vi "Machine_Etat_M1.vi"() -> ()   [LabVIEW 2017]
uses:
  Commande 1.ctl
  <vilib>/Platform/TimedLoop/XDataNode/timing_clust.ctl
  <vilib>/Platform/TimedLoop/XDataNode/nitl_modes.ctl
  <vilib>/Platform/TimedLoop/XDataNode/wakeup.ctl
  <vilib>/myRIO/Instrument Drivers/Onboard IO/DIO/typedefs/DIO Reference.ctl
  <vilib>/myRIO/Common/Instrument Driver Framework/Utilities/typedefs/myRIO Generic Hardware Reference.ctl
  <vilib>/myRIO/Common/Instrument Driver Framework/Utilities/typedefs/Hardware Version Enum.ctl
  <vilib>/myRIO/Common/Instrument Driver Framework/Utilities/typedefs/myRIO v1.0 Reference.ctl
  <vilib>/myRIO/Common/Instrument Driver Framework/Utilities/typedefs/Generic FPGA Reference.ctl
  <vilib>/myRIO/Common/Instrument Driver Framework/myRIO v1.0/DIO/typedefs/DIO Channels List.ctl
  <vilib>/myRIO/Common/Instrument Driver Framework/myRIO v1.0/DIO/typedefs/DIO Channels Enum.ctl
  <vilib>/userdefined/High Color/nirio_resource_hc.ctl
  enum_bras.ctl
  <vilib>/myRIO/Common/Instrument Driver Framework/Utilities/vis/Is FPGA Ref Available.vi
  <vilib>/myRIO/Common/Instrument Driver Framework/myRIO v1.0/DIO/vis/myRIO v1.1 Open DIO.vi
  <vilib>/myRIO/Instrument Drivers/Onboard IO/DIO/vis/Write.vi
  <vilib>/myRIO/Common/Instrument Driver Framework/Utilities/vis/Validate Channels.vi
  <vilib>/myRIO/Common/Instrument Driver Framework/myRIO v1.0/DIO/vis/myRIO v1.0 Reserve DIO.vi
  <vilib>/myRIO/Common/Instrument Driver Framework/myRIO v1.0/Resource Manager/vis/myRIO v1.0 Reserve Channel List.vi
  <vilib>/myRIO/Common/Instrument Driver Framework/myRIO v1.0/DIO/vis/myRIO v1.0 Build MUX Configuration DIO.vi
  <vilib>/myRIO/Common/Instrument Driver Framework/myRIO v1.0/Resource Manager/vis/myRIO v1.0 Reserve Channel.vi
  <vilib>/myRIO/Common/Instrument Driver Framework/myRIO v1.0/Resource Manager/vis/myRIO v1.0 Unreserve Channel.vi
  <vilib>/myRIO/Common/Instrument Driver Framework/myRIO v1.0/Resource Manager/vis/myRIO v1.0 Create Configuration List.vi
  <vilib>/myRIO/Common/Instrument Driver Framework/myRIO v1.0/Resource Manager/vis/myRIO v1.0 Build Mutex Name.vi
  <vilib>/Utility/VariantDataType/GetNumericInfo.vi
  <vilib>/Utility/error.llb/Error Cluster From Error Code.vi
  <vilib>/myRIO/Common/Instrument Driver Framework/myRIO v1.0/myRIO v1.1 Open.vi
  <vilib>/myRIO/Common/Instrument Driver Framework/Utilities/vis/IO Manager.vi
  <vilib>/myRIO/Common/Instrument Driver Framework/Utilities/vis/Configuration Manager.vi
  <vilib>/myRIO/Common/Instrument Driver Framework/myRIO v1.0/Resource Manager/vis/myRIO v1.0 Configure IO.vi
  <vilib>/myRIO/Common/Instrument Driver Framework/myRIO v1.0/myRIO v1.0 Close.vi
  <vilib>/myRIO/Common/Instrument Driver Framework/myRIO v1.0/DIO/vis/myRIO v1.0 Write DIO.vi
  <vilib>/Platform/TimedLoop/XDataNode/XDataNode.xnode
  <vilib>/myRIO/Express VI/Onboard Devices/LED/LED Express VI.xnode
  <vilib>/myRIO/Instrument Drivers/Onboard IO/DIO/vis/myRIO DIO Open.xnode
  <vilib>/Platform/TimedLoop/XDataNode/XDNodeRunTimeDep.lvlib
  <vilib>/myRIO/Instrument Drivers/Onboard IO/DIO/DIO.lvlib
panel:
  out "Erreur":errorcluster
  out "Vert : dévi à droite 2":bool
  out "Graphe déroulant 2":u32(graph)
  out "x > y ? 2":bool[](array[boolean])
  out "Cluster 3":T1
  out "4 LED droite 2":bool[](array[boolean])
  out "4 LED gauche 2":bool[](array[boolean])
  out "droite 2":u32
  out "gauche 2":u32
  out "Énum 2":T2
  out "seuil":u32
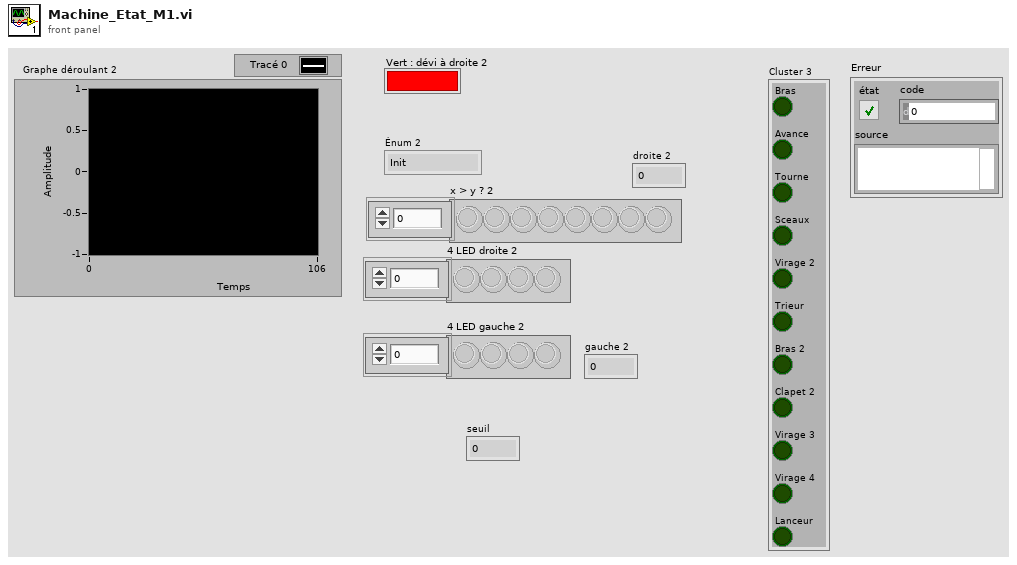
[diagram p1: front panel]
types:
  T1 = typedef "Voyant machine d'état.ctl" = cluster{"Bras":bool, "Avance":bool, "Tourne":bool, "Sceaux":bool, "Virage 2":bool, "Trieur":bool, "Bras 2":bool, "Clapet 2":bool, "Virage 3":bool, "Virage 4":bool, "Lanceur":bool}
  T2 = typedef "Commande 1.ctl" = enum16{"Init", "Bras", "Clapet 1", "Virage 1", "Sceaux 0", "Sceaux 1", "Sceaux 2", "Sceaux 3", "Sceaux 4", "Virage 2", "Recule", "Trieur", "Bras 2", "Intersection", "Clapet 2", "Virage 3", "Virage 4", "Avance", "Lanceur", "End"}
  T3 = typedef "XDNodeRunTimeDep.lvlib/timing_clust.ctl" = cluster{"Expected End [f-1]":u64, "Actual End [f-1]":u64, "Finished Late? [f-1]":bool, "Expected End [i-1]":u64, "Actual End [i-1]":u64, "Finished Late? [i-1]":bool, "Expected Start [i]":u64, "Actual Start [i]":u64, "Expected Start [f]":u64, "Actual Start [f]":u64, "Source Name":string, "Structure Name":string, "Period":i64, "Deadline":i64, "Offset":i64, "Start":i64, "Priority":i32, "Timeout":i32, "Mode":T4, "Wakeup Reason":T5, "Error":errorcluster, "Source Type":string, "Secondary Source Type":string, "Global End Time":u64, "Global Start Time":u64, "Frame Duration":u64, "Iteration Duration":u64, "Assigned CPU":i32, "I/O Scan Engine Mode":u32}
  T4 = typedef "XDNodeRunTimeDep.lvlib/nitl_modes.ctl" = enum32{"No Change", "Process missed periods, maintain original phase", "Discard missed periods, maintain original phase", "Process missed periods, ignore original phase", "Discard missed periods, ignore original phase"}
  T5 = typedef "XDNodeRunTimeDep.lvlib/wakeup.ctl" = enum32{"Normal", "Aborted", "Asynchronous wakeup", "Timing source error", "Timed loop error", "Timeout"}
  T6 = typedef "DIO.lvlib/DIO Reference.ctl" = cluster{"myRIO Reference":T7, "DIO Channels List":T11}
  T7 = typedef "myRIO Generic Hardware Reference.ctl" = cluster{"myRIO Model":T8, "myRIO Hardware Reference":T9}
  T8 = typedef "Hardware Version Enum.ctl" = enum16{"Unknown", "myRIO-1900", "myRIO-1950", "roboRIO", "NI ELVIS RIO CM"}
  T9 = typedef "myRIO v1.0 Reference.ctl" = cluster{"Generic FPGA Reference":T10, "Allow multiple opens":bool}
  T10 = typedef "Generic FPGA Reference.ctl" = refnum<k20>
  T11 = typedef "DIO Channels List.ctl" = T12[]
  T12 = typedef "DIO Channels Enum.ctl" = enum16{"Not Connected", "C/DIO0", "C/DIO1", "C/DIO2", "C/DIO3", "C/DIO4", "C/DIO5", "C/DIO6", "C/DIO7", "A/DIO0", "A/DIO1", "A/DIO2", "A/DIO3", "A/DIO4", "A/DIO5", "A/DIO6", "A/DIO7", "A/DIO8", "A/DIO9", "A/DIO10", "A/DIO11", "A/DIO12", "A/DIO13", "A/DIO14", "A/DIO15", "B/DIO0", "B/DIO1", "B/DIO2", "B/DIO3", "B/DIO4", "B/DIO5", "B/DIO6", "B/DIO7", "B/DIO8", "B/DIO9", "B/DIO10", "B/DIO11", "B/DIO12", "B/DIO13", "B/DIO14", "B/DIO15", "LED0", "LED1", "LED2", "LED3", "Button0", "DIO/DIO0", "DIO/DIO1", "DIO/DIO2", "DIO/DIO3", "DIO/DIO4", "DIO/DIO5", "DIO/DIO6", "DIO/DIO7", "DIO/DIO8", "DIO/DIO9", "SPI/CS0", "SPI/CS1", "SPI/CS2", "SPI/CS3", "LED RADIO (Green)", "LED RADIO (Red)", "LED COMM (Green)", "LED COMM (Red)", "LED MODE (Green)", "LED MODE (Red)"}
  T13 = typedef "nirio_resource_hc.ctl" = tag
  T14 = typedef "enum_bras.ctl" = enum16{"Depart Bras", "Clapet Bras", "Inactif Bras", "Seaux Bras"}
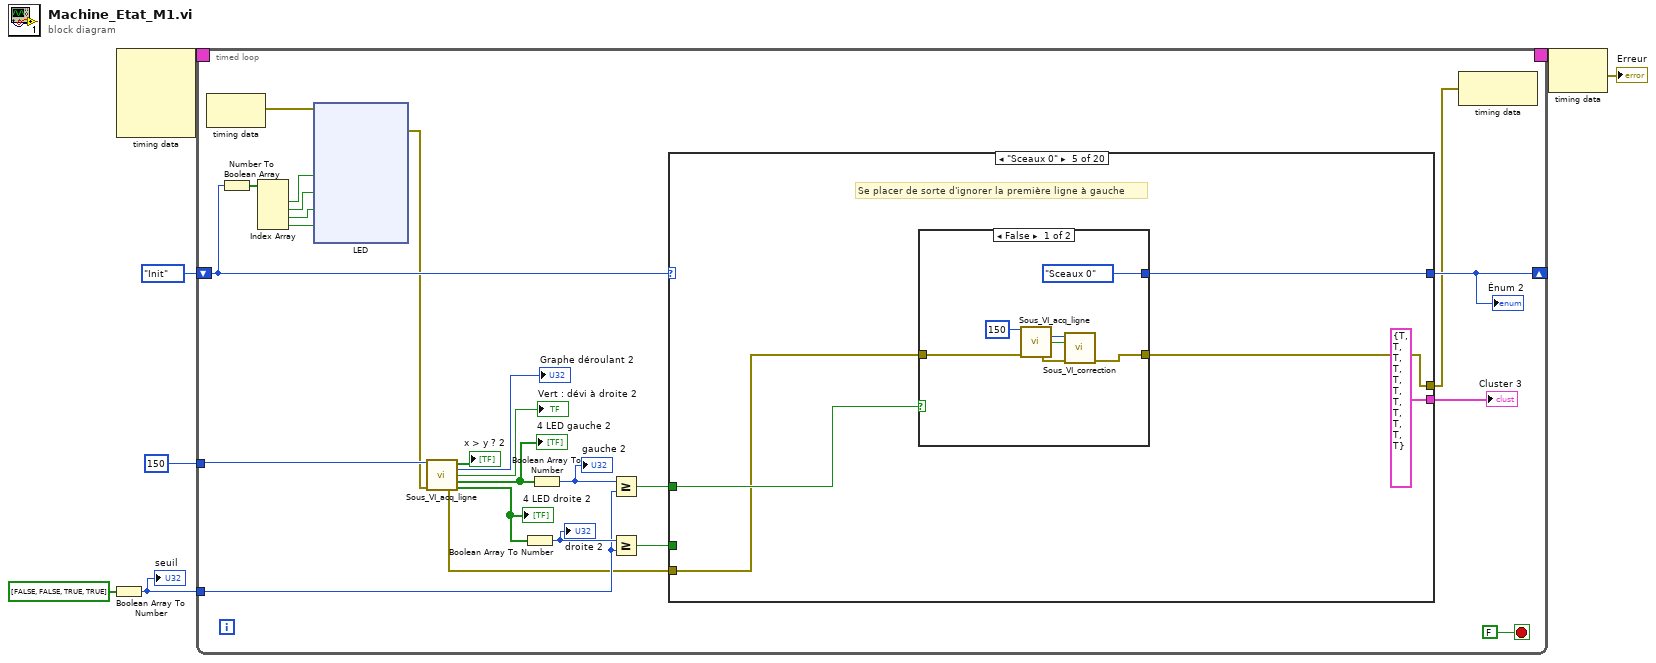
[diagram p0: block diagram]
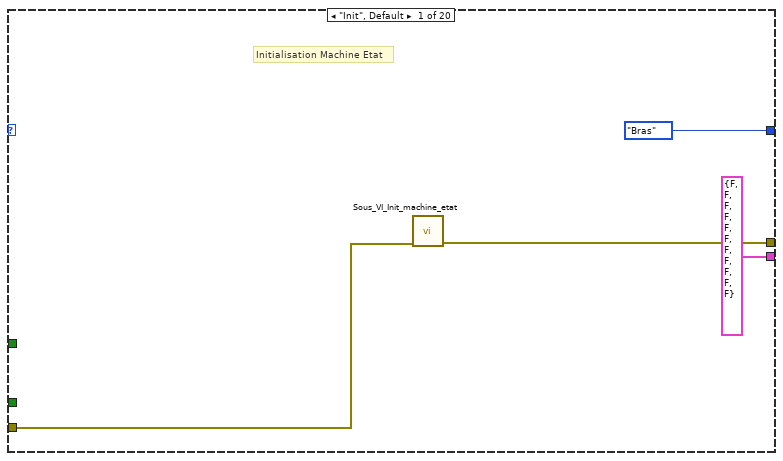
[diagram p2: hidden frame]
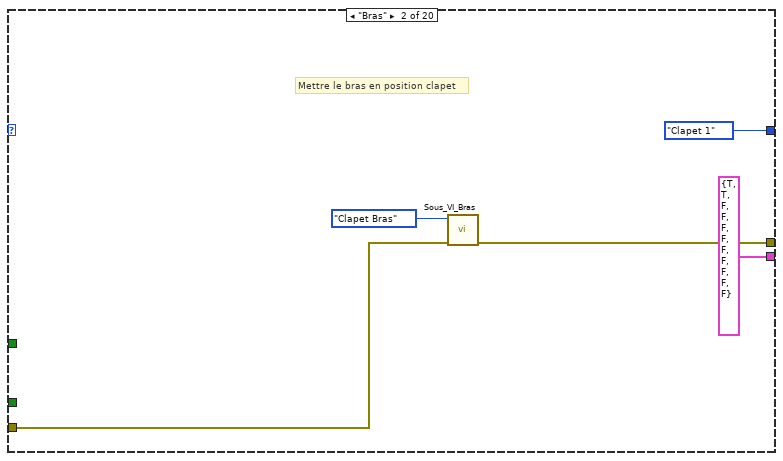
[diagram p3: hidden frame]
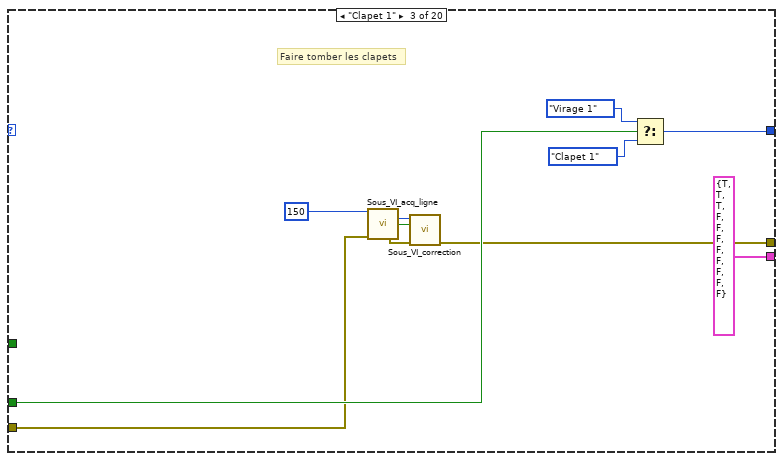
[diagram p4: hidden frame]
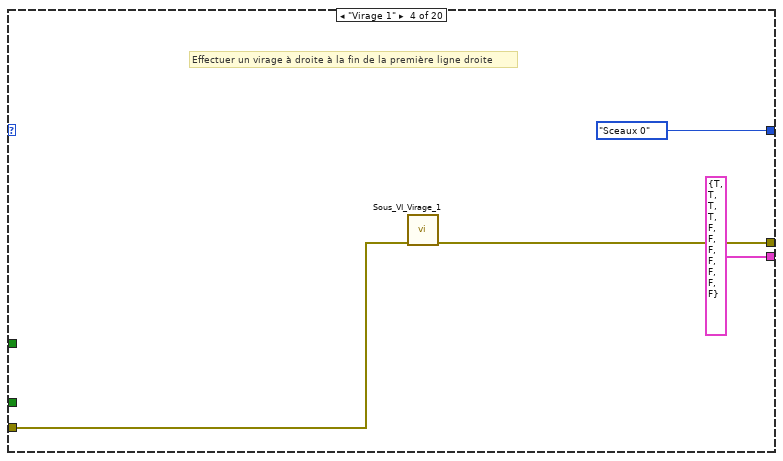
[diagram p5: hidden frame]
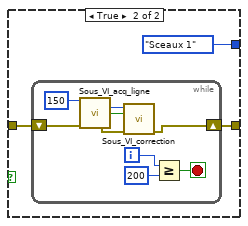
[diagram p6: hidden frame]
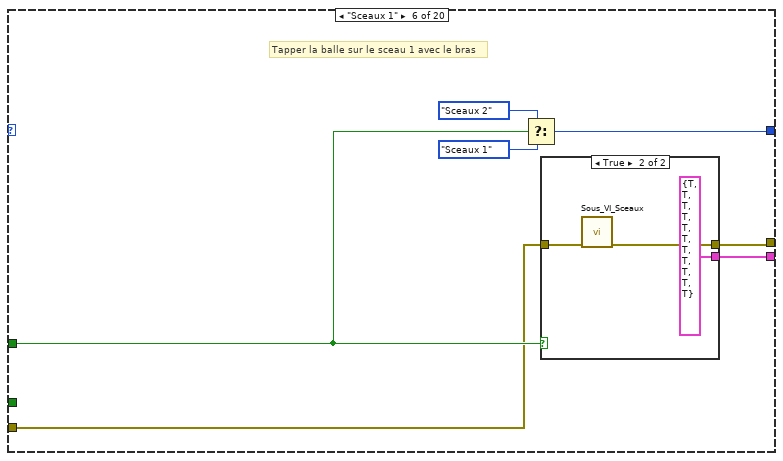
[diagram p7: hidden frame]
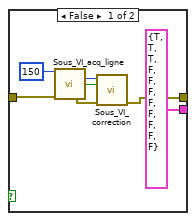
[diagram p8: hidden frame]
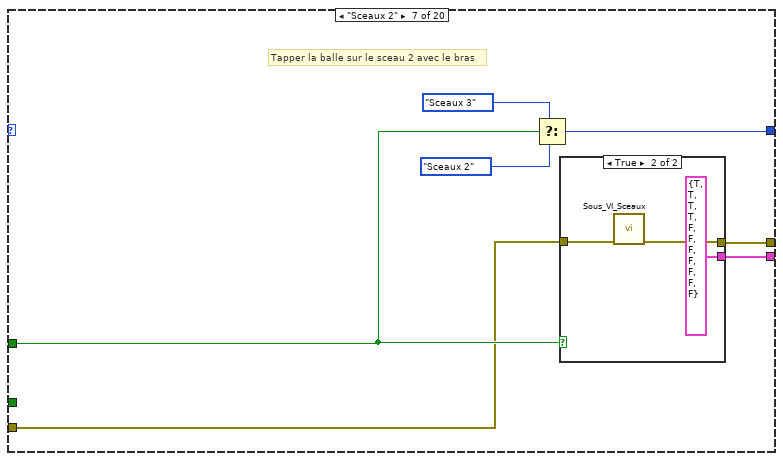
[diagram p9: hidden frame]
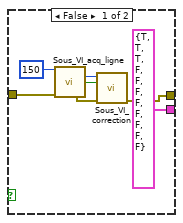
[diagram p10: hidden frame]
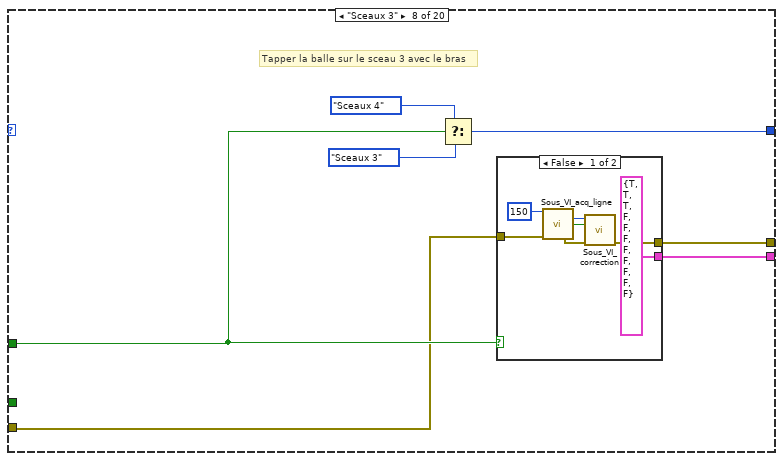
[diagram p11: hidden frame]
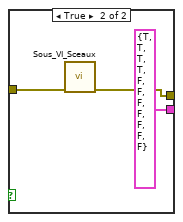
[diagram p12: hidden frame]
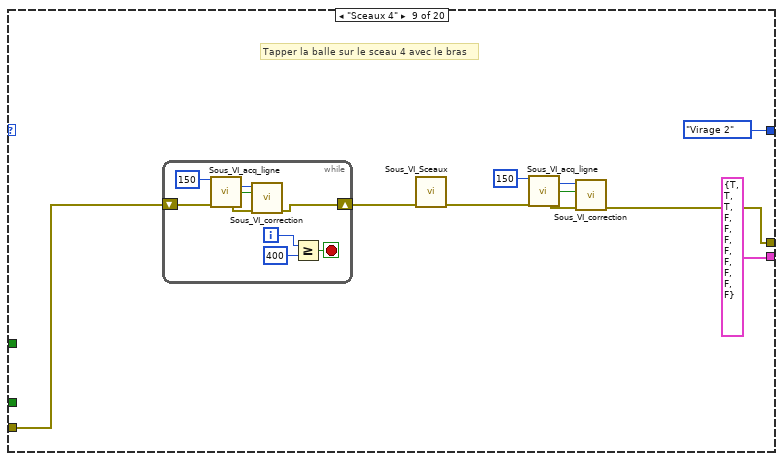
[diagram p13: hidden frame]
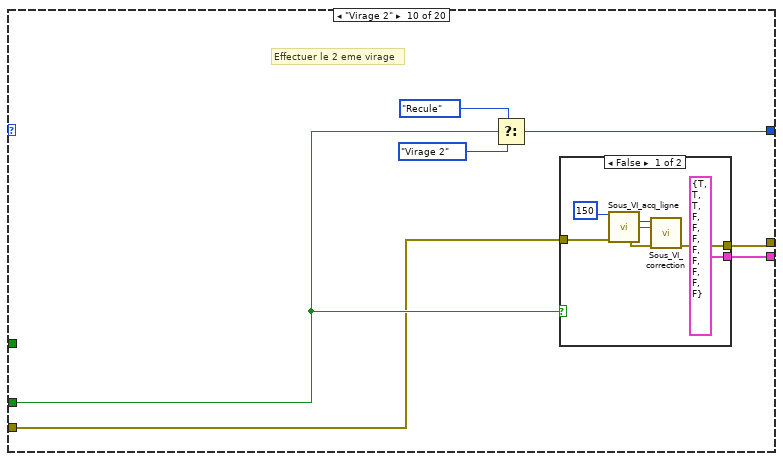
[diagram p14: hidden frame]
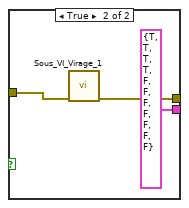
[diagram p15: hidden frame]
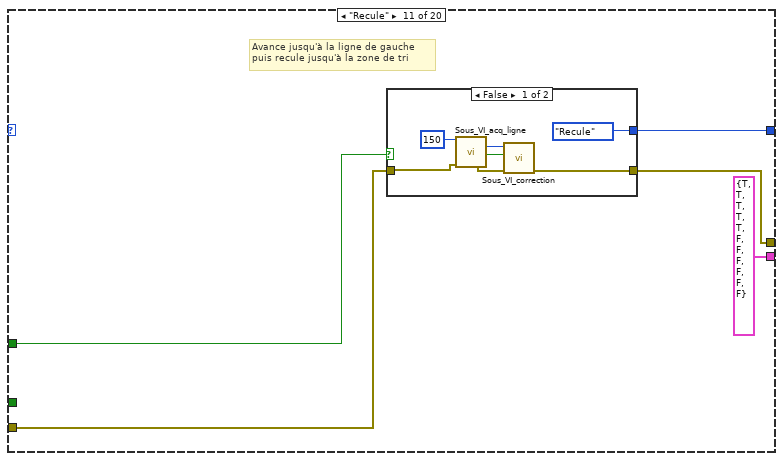
[diagram p16: hidden frame]
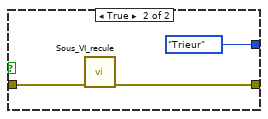
[diagram p17: hidden frame]
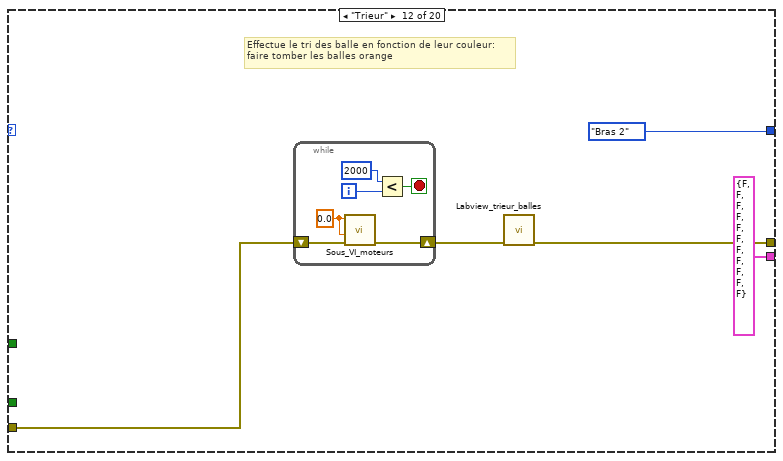
[diagram p18: hidden frame]
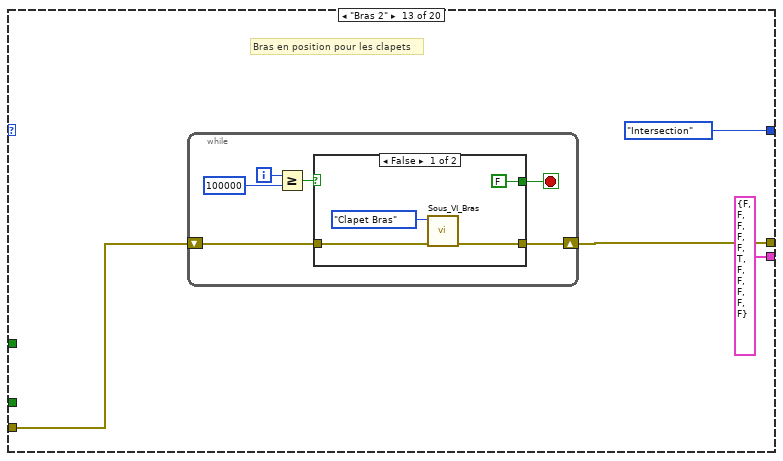
[diagram p19: hidden frame]
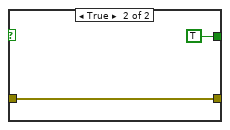
[diagram p20: hidden frame]
diagram:
  n1 = Boolean Array To Number(Boolean array=bool[] [FALSE, FALSE, TRUE, TRUE] ("x < y ? 2")) -> (number=w3:u32)
  "seuil" <- w3
  n2 = node-c288() -> (w6:T3)  [unwired: 4 in]
  n3 = timed-loop {
    tunnel: 150 ("value") -> [w26]
    shift-right: [w31] -> _
    shift-left: Commande_1."Init" -> [w18]
    tunnel: w3 -> [w20]
    timing: w6 -> [_]
    timing-out: [_] -> w5
    stop <- FALSE stop-if-true
    n4 = node-c288() -> (w11:errorcluster)  [unwired: 1 in]
    n5 = Number To Boolean Array(number=w18) -> (Boolean array=w17:bool[])
    n6 = Index Array(array=w17) -> (element #1=w16:bool, element #2=w15:bool, element #3=w12:bool, element #4=w14:bool)  [unwired: 4 in]
    n7 = xnode "LED"("LED0"=w16, "LED1"=w15, "LED2"=w12, "LED3"=w14, "error in (no error)"=w11) -> ("error out"=w10:errorcluster)
    n8 = call "Sous_VI_acq_ligne.vi"("Seuil"=w26, "error in (no error)"=w10) -> ("x > y ?"=→"x > y ? 2":bool[], "Décalage"=→"Graphe déroulant 2":u32, "G/D ?"=→"Vert : dévi à droite 2":bool, "4 LED gauches"=w23:bool[], "error out"=w9:errorcluster, "4 LED droite"=w22:bool[])  [unwired: 8 in]
    "4 LED droite 2" <- w22
    "4 LED gauche 2" <- w23
    n9 = Boolean Array To Number(Boolean array=w22) -> (number=w21:u32)
    "droite 2" <- w21
    n10 = Boolean Array To Number(Boolean array=w23) -> (number=w19:u32)
    "gauche 2" <- w19
    n11 = Greater Or Equal?(x=w19, y=w20) -> (x >= y?=w29:bool)
    n12 = Greater Or Equal?(x=w21, y=w20) -> (x >= y?=w30:bool)
    n13 = case shown="\"Sceaux 0\"" w18 {
      tunnel: [Commande_1."Bras" Commande_1."Clapet 1" w92 Commande_1."Sceaux 0" w103 w127 w144 w160 Commande_1."Virage 2" w196 w212 Commande_1."Bras 2" Commande_1."Intersection" w257 w268 Commande_1."Avance" w305 Commande_1."Lanceur" Commande_1."End" Commande_1."End"] -> w31
      tunnel: w30 -> [_ _ w91 _ _ _ _ _ _ w195 _ _ _ _ w267 _ w304 _ _ _]
      tunnel: [T1 {"Bras"=FALSE, "Avance"=FALSE, "Tourne"=FALSE, "Sceaux"=FALSE, "Virage 2"=FALSE, "Trieur"=FALSE, "Bras 2"=FALSE, "Clapet 2"=FALSE, "Virage 3"=FALSE, "Virage 4"=FALSE, "Lanceur"=FALSE} ("Cluster 2") T1 {"Bras"=TRUE, "Avance"=TRUE, "Tourne"=FALSE, "Sceaux"=FALSE, "Virage 2"=FALSE, "Trieur"=FALSE, "Bras 2"=FALSE, "Clapet 2"=FALSE, "Virage 3"=FALSE, "Virage 4"=FALSE, "Lanceur"=FALSE} ("Cluster 2") T1 {"Bras"=TRUE, "Avance"=TRUE, "Tourne"=TRUE, "Sceaux"=FALSE, "Virage 2"=FALSE, "Trieur"=FALSE, "Bras 2"=FALSE, "Clapet 2"=FALSE, "Virage 3"=FALSE, "Virage 4"=FALSE, "Lanceur"=FALSE} ("Cluster 2") T1 {"Bras"=TRUE, "Avance"=TRUE, "Tourne"=TRUE, "Sceaux"=TRUE, "Virage 2"=FALSE, "Trieur"=FALSE, "Bras 2"=FALSE, "Clapet 2"=FALSE, "Virage 3"=FALSE, "Virage 4"=FALSE, "Lanceur"=FALSE} ("Cluster 2") T1 {"Bras"=TRUE, "Avance"=TRUE, "Tourne"=TRUE, "Sceaux"=TRUE, "Virage 2"=TRUE, "Trieur"=TRUE, "Bras 2"=TRUE, "Clapet 2"=TRUE, "Virage 3"=TRUE, "Virage 4"=TRUE, "Lanceur"=TRUE} ("Cluster 2") w126 w146 w163 T1 {"Bras"=TRUE, "Avance"=TRUE, "Tourne"=TRUE, "Sceaux"=FALSE, "Virage 2"=FALSE, "Trieur"=FALSE, "Bras 2"=FALSE, "Clapet 2"=FALSE, "Virage 3"=FALSE, "Virage 4"=FALSE, "Lanceur"=FALSE} ("Cluster 2") w199 T1 {"Bras"=TRUE, "Avance"=TRUE, "Tourne"=TRUE, "Sceaux"=TRUE, "Virage 2"=TRUE, "Trieur"=FALSE, "Bras 2"=FALSE, "Clapet 2"=FALSE, "Virage 3"=FALSE, "Virage 4"=FALSE, "Lanceur"=FALSE} ("Cluster 2") T1 {"Bras"=FALSE, "Avance"=FALSE, "Tourne"=FALSE, "Sceaux"=FALSE, "Virage 2"=FALSE, "Trieur"=FALSE, "Bras 2"=FALSE, "Clapet 2"=FALSE, "Virage 3"=FALSE, "Virage 4"=FALSE, "Lanceur"=FALSE} ("Cluster 2") T1 {"Bras"=FALSE, "Avance"=FALSE, "Tourne"=FALSE, "Sceaux"=FALSE, "Virage 2"=FALSE, "Trieur"=TRUE, "Bras 2"=FALSE, "Clapet 2"=FALSE, "Virage 3"=FALSE, "Virage 4"=FALSE, "Lanceur"=FALSE} ("Cluster 2") T1 {"Bras"=FALSE, "Avance"=FALSE, "Tourne"=FALSE, "Sceaux"=FALSE, "Virage 2"=FALSE, "Trieur"=TRUE, "Bras 2"=TRUE, "Clapet 2"=FALSE, "Virage 3"=FALSE, "Virage 4"=FALSE, "Lanceur"=FALSE} ("Cluster 2") T1 {"Bras"=FALSE, "Avance"=FALSE, "Tourne"=FALSE, "Sceaux"=FALSE, "Virage 2"=FALSE, "Trieur"=TRUE, "Bras 2"=TRUE, "Clapet 2"=FALSE, "Virage 3"=FALSE, "Virage 4"=FALSE, "Lanceur"=FALSE} ("Cluster 2") T1 {"Bras"=FALSE, "Avance"=FALSE, "Tourne"=FALSE, "Sceaux"=FALSE, "Virage 2"=FALSE, "Trieur"=TRUE, "Bras 2"=TRUE, "Clapet 2"=TRUE, "Virage 3"=TRUE, "Virage 4"=FALSE, "Lanceur"=FALSE} ("Cluster 2") T1 {"Bras"=FALSE, "Avance"=FALSE, "Tourne"=FALSE, "Sceaux"=FALSE, "Virage 2"=FALSE, "Trieur"=FALSE, "Bras 2"=TRUE, "Clapet 2"=TRUE, "Virage 3"=TRUE, "Virage 4"=TRUE, "Lanceur"=FALSE} ("Cluster 2") T1 {"Bras"=FALSE, "Avance"=FALSE, "Tourne"=FALSE, "Sceaux"=FALSE, "Virage 2"=FALSE, "Trieur"=TRUE, "Bras 2"=TRUE, "Clapet 2"=TRUE, "Virage 3"=TRUE, "Virage 4"=TRUE, "Lanceur"=FALSE} ("Cluster 2") T1 {"Bras"=FALSE, "Avance"=FALSE, "Tourne"=FALSE, "Sceaux"=FALSE, "Virage 2"=FALSE, "Trieur"=FALSE, "Bras 2"=TRUE, "Clapet 2"=TRUE, "Virage 3"=TRUE, "Virage 4"=TRUE, "Lanceur"=TRUE} ("Cluster 2") T1 {"Bras"=FALSE, "Avance"=FALSE, "Tourne"=FALSE, "Sceaux"=FALSE, "Virage 2"=FALSE, "Trieur"=FALSE, "Bras 2"=FALSE, "Clapet 2"=FALSE, "Virage 3"=FALSE, "Virage 4"=FALSE, "Lanceur"=FALSE} ("Cluster 2")] -> w25
      tunnel: w29 -> [_ _ _ _ w102 w125 w143 w159 _ _ w213 _ _ w258 _ _ _ _ _ _]
      tunnel: w9 -> [w75 w80 w84 w95 w100 w124 w141 w158 w181 w194 w211 w227 w237 w252 w263 w277 w298 w309 w313 w317]
      tunnel: [w76 w79 w86 w96 w99 w123 w140 w157 w178 w193 w210 w225 w236 w254 w265 w274 w300 w310 w314 w317] -> w8
      frame "Init", Default {
        # "Initialisation Machine Etat"
        n14 = call "Sous_VI_Init_machine_etat.vi"("error in (no error)"=w75) -> ("error out"=w76:errorcluster)  [unwired: 10 in]
      }
      frame "Bras" {
        # "Mettre le bras en position clapet"
        n15 = call "Sous_VI_Bras.vi"("error in (no error)"=w80, "Enum bras"=enum_bras."Clapet Bras") -> ("error out"=w79:errorcluster)  [unwired: 9 in]
      }
      frame "Clapet 1" {
        # "Faire tomber les clapets"
        n16 = call "Sous_VI_acq_ligne.vi"("Seuil"=150, "error in (no error)"=w84) -> ("Décalage"=w89:u32, "G/D ?"=w87:bool, "error out"=w85:errorcluster)  [unwired: 8 in, 3 out]
        n17 = call "Sous_VI_correction.vi"("error in (no error)"=w85, "G/D ?"=w87, "Décalage"=w89) -> ("error out"=w86:errorcluster)  [unwired: 8 in]
        n18 = Select(t=Commande_1."Virage 1", s=w91, f=Commande_1."Clapet 1") -> (s? t:f=w92:T2)
      }
      frame "Virage 1" {
        # "Effectuer un virage à droite à la fin de la première ligne droite"
        n19 = call "Sous_VI_Virage_1.vi"("error in (no error)"=w95) -> ("error out"=w96:errorcluster)  [unwired: 10 in]
      }
      frame "Sceaux 0" {
        # "Se placer de sorte d'ignorer la première ligne à gauche"
        n20 = case shown="False" w102 {
          tunnel: [Commande_1."Sceaux 0" Commande_1."Sceaux 1"] -> w103
          tunnel: w100 -> [w104 w112]
          tunnel: [w106 w111] -> w99
          frame False {
            n21 = call "Sous_VI_acq_ligne.vi"("Seuil"=150, "error in (no error)"=w104) -> ("Décalage"=w109:u32, "G/D ?"=w107:bool, "error out"=w105:errorcluster)  [unwired: 8 in, 3 out]
            n22 = call "Sous_VI_correction.vi"("error in (no error)"=w105, "G/D ?"=w107, "Décalage"=w109) -> ("error out"=w106:errorcluster)  [unwired: 8 in]
          }
          frame True {
            n23 = while {
              shift-right: [w114] -> w111
              shift-left: w112 -> [w116]
              i -> [w122]
              stop <- w118 stop-if-true
              n24 = call "Sous_VI_acq_ligne.vi"("Seuil"=150, "error in (no error)"=w116) -> ("Décalage"=w120:u32, "G/D ?"=w117:bool, "error out"=w115:errorcluster)  [unwired: 8 in, 3 out]
              n25 = call "Sous_VI_correction.vi"("error in (no error)"=w115, "G/D ?"=w117, "Décalage"=w120) -> ("error out"=w114:errorcluster)  [unwired: 8 in]
              n26 = Greater Or Equal?(x=w122, y=200) -> (x >= y?=w118:bool)
            }
          }
        }
      }
      frame "Sceaux 1" {
        # "Tapper la balle sur le sceau 1 avec le bras"
        n27 = Select(t=Commande_1."Sceaux 2", s=w125, f=Commande_1."Sceaux 1") -> (s? t:f=w127:T2)
        n28 = case shown="True" w125 {
          tunnel: [T1 {"Bras"=TRUE, "Avance"=TRUE, "Tourne"=TRUE, "Sceaux"=FALSE, "Virage 2"=FALSE, "Trieur"=FALSE, "Bras 2"=FALSE, "Clapet 2"=FALSE, "Virage 3"=FALSE, "Virage 4"=FALSE, "Lanceur"=FALSE} ("Cluster 2") T1 {"Bras"=TRUE, "Avance"=TRUE, "Tourne"=TRUE, "Sceaux"=TRUE, "Virage 2"=TRUE, "Trieur"=TRUE, "Bras 2"=TRUE, "Clapet 2"=TRUE, "Virage 3"=TRUE, "Virage 4"=TRUE, "Lanceur"=TRUE} ("Cluster 2")] -> w126
          tunnel: w124 -> [w132 w138]
          tunnel: [w130 w137] -> w123
          frame False {
            n29 = call "Sous_VI_acq_ligne.vi"("Seuil"=150, "error in (no error)"=w132) -> ("Décalage"=w135:u32, "G/D ?"=w133:bool, "error out"=w131:errorcluster)  [unwired: 8 in, 3 out]
            n30 = call "Sous_VI_correction.vi"("error in (no error)"=w131, "G/D ?"=w133, "Décalage"=w135) -> ("error out"=w130:errorcluster)  [unwired: 8 in]
          }
          frame True {
            n31 = call "Sous_VI_Sceaux.vi"("error in (no error)"=w138) -> ("error out"=w137:errorcluster)  [unwired: 10 in]
          }
        }
      }
      frame "Sceaux 2" {
        # "Tapper la balle sur le sceau 2 avec le bras"
        n32 = Select(t=Commande_1."Sceaux 3", s=w143, f=Commande_1."Sceaux 2") -> (s? t:f=w144:T2)
        n33 = case shown="True" w143 {
          tunnel: [T1 {"Bras"=TRUE, "Avance"=TRUE, "Tourne"=TRUE, "Sceaux"=FALSE, "Virage 2"=FALSE, "Trieur"=FALSE, "Bras 2"=FALSE, "Clapet 2"=FALSE, "Virage 3"=FALSE, "Virage 4"=FALSE, "Lanceur"=FALSE} ("Cluster 2") T1 {"Bras"=TRUE, "Avance"=TRUE, "Tourne"=TRUE, "Sceaux"=TRUE, "Virage 2"=FALSE, "Trieur"=FALSE, "Bras 2"=FALSE, "Clapet 2"=FALSE, "Virage 3"=FALSE, "Virage 4"=FALSE, "Lanceur"=FALSE} ("Cluster 2")] -> w146
          tunnel: w141 -> [w149 w155]
          tunnel: [w147 w154] -> w140
          frame False {
            n34 = call "Sous_VI_acq_ligne.vi"("Seuil"=150, "error in (no error)"=w149) -> ("Décalage"=w152:u32, "G/D ?"=w150:bool, "error out"=w148:errorcluster)  [unwired: 8 in, 3 out]
            n35 = call "Sous_VI_correction.vi"("error in (no error)"=w148, "G/D ?"=w150, "Décalage"=w152) -> ("error out"=w147:errorcluster)  [unwired: 8 in]
          }
          frame True {
            n36 = call "Sous_VI_Sceaux.vi"("error in (no error)"=w155) -> ("error out"=w154:errorcluster)  [unwired: 10 in]
          }
        }
      }
      frame "Sceaux 3" {
        # "Tapper la balle sur le sceau 3 avec le bras"
        n37 = Select(t=Commande_1."Sceaux 4", s=w159, f=Commande_1."Sceaux 3") -> (s? t:f=w160:T2)
        n38 = case shown="False" w159 {
          tunnel: [T1 {"Bras"=TRUE, "Avance"=TRUE, "Tourne"=TRUE, "Sceaux"=FALSE, "Virage 2"=FALSE, "Trieur"=FALSE, "Bras 2"=FALSE, "Clapet 2"=FALSE, "Virage 3"=FALSE, "Virage 4"=FALSE, "Lanceur"=FALSE} ("Cluster 2") T1 {"Bras"=TRUE, "Avance"=TRUE, "Tourne"=TRUE, "Sceaux"=TRUE, "Virage 2"=FALSE, "Trieur"=FALSE, "Bras 2"=FALSE, "Clapet 2"=FALSE, "Virage 3"=FALSE, "Virage 4"=FALSE, "Lanceur"=FALSE} ("Cluster 2")] -> w163
          tunnel: w158 -> [w166 w172]
          tunnel: [w164 w171] -> w157
          frame False {
            n39 = call "Sous_VI_acq_ligne.vi"("Seuil"=150, "error in (no error)"=w166) -> ("Décalage"=w169:u32, "G/D ?"=w167:bool, "error out"=w165:errorcluster)  [unwired: 8 in, 3 out]
            n40 = call "Sous_VI_correction.vi"("error in (no error)"=w165, "G/D ?"=w167, "Décalage"=w169) -> ("error out"=w164:errorcluster)  [unwired: 8 in]
          }
          frame True {
            n41 = call "Sous_VI_Sceaux.vi"("error in (no error)"=w172) -> ("error out"=w171:errorcluster)  [unwired: 10 in]
          }
        }
      }
      frame "Sceaux 4" {
        # "Tapper la balle sur le sceau 4 avec le bras"
        n42 = while {
          shift-right: [w184] -> w180
          shift-left: w181 -> [w186]
          i -> [w192]
          stop <- w188 stop-if-true
          n43 = call "Sous_VI_acq_ligne.vi"("Seuil"=150, "error in (no error)"=w186) -> ("Décalage"=w190:u32, "G/D ?"=w187:bool, "error out"=w185:errorcluster)  [unwired: 8 in, 3 out]
          n44 = call "Sous_VI_correction.vi"("error in (no error)"=w185, "G/D ?"=w187, "Décalage"=w190) -> ("error out"=w184:errorcluster)  [unwired: 8 in]
          n45 = Greater Or Equal?(x=w192, y=400) -> (x >= y?=w188:bool)
        }
        n46 = call "Sous_VI_Sceaux.vi"("error in (no error)"=w180) -> ("error out"=w179:errorcluster)  [unwired: 10 in]
        n47 = call "Sous_VI_acq_ligne.vi"("Seuil"=150, "error in (no error)"=w179) -> ("Décalage"=w177:u32, "G/D ?"=w175:bool, "error out"=w174:errorcluster)  [unwired: 8 in, 3 out]
        n48 = call "Sous_VI_correction.vi"("error in (no error)"=w174, "G/D ?"=w175, "Décalage"=w177) -> ("error out"=w178:errorcluster)  [unwired: 8 in]
      }
      frame "Virage 2" {
        # "Effectuer le 2 eme virage"
        n49 = Select(t=Commande_1."Recule", s=w195, f=Commande_1."Virage 2") -> (s? t:f=w196:T2)
        n50 = case shown="False" w195 {
          tunnel: [T1 {"Bras"=TRUE, "Avance"=TRUE, "Tourne"=TRUE, "Sceaux"=FALSE, "Virage 2"=FALSE, "Trieur"=FALSE, "Bras 2"=FALSE, "Clapet 2"=FALSE, "Virage 3"=FALSE, "Virage 4"=FALSE, "Lanceur"=FALSE} ("Cluster 2") T1 {"Bras"=TRUE, "Avance"=TRUE, "Tourne"=TRUE, "Sceaux"=TRUE, "Virage 2"=FALSE, "Trieur"=FALSE, "Bras 2"=FALSE, "Clapet 2"=FALSE, "Virage 3"=FALSE, "Virage 4"=FALSE, "Lanceur"=FALSE} ("Cluster 2")] -> w199
          tunnel: w194 -> [w202 w208]
          tunnel: [w200 w207] -> w193
          frame False {
            n51 = call "Sous_VI_acq_ligne.vi"("Seuil"=150, "error in (no error)"=w202) -> ("Décalage"=w205:u32, "G/D ?"=w203:bool, "error out"=w201:errorcluster)  [unwired: 8 in, 3 out]
            n52 = call "Sous_VI_correction.vi"("error in (no error)"=w201, "G/D ?"=w203, "Décalage"=w205) -> ("error out"=w200:errorcluster)  [unwired: 8 in]
          }
          frame True {
            n53 = call "Sous_VI_Virage_1.vi"("error in (no error)"=w208) -> ("error out"=w207:errorcluster)  [unwired: 10 in]
          }
        }
      }
      frame "Recule" {
        # "Avance jusqu'à la ligne de gauche \npuis recule jusqu'à la zone de tri"
        n54 = case shown="False" w213 {
          tunnel: [Commande_1."Recule" Commande_1."Trieur"] -> w212
          tunnel: w211 -> [w215 w223]
          tunnel: [w216 w222] -> w210
          frame False {
            n55 = call "Sous_VI_acq_ligne.vi"("Seuil"=150, "error in (no error)"=w215) -> ("Décalage"=w219:u32, "G/D ?"=w218:bool, "error out"=w217:errorcluster)  [unwired: 8 in, 3 out]
            n56 = call "Sous_VI_correction.vi"("error in (no error)"=w217, "G/D ?"=w218, "Décalage"=w219) -> ("error out"=w216:errorcluster)  [unwired: 8 in]
          }
          frame True {
            n57 = call "Sous_VI_recule.vi"("error in (no error)"=w223) -> ("error out"=w222:errorcluster)  [unwired: 10 in]
          }
        }
      }
      frame "Trieur" {
        # "Effectue le tri des balle en fonction de leur couleur:\nfaire tomber les balles orange"
        n58 = while {
          shift-right: [w230] -> w226
          shift-left: w227 -> [w231]
          i -> [w235]
          stop <- w233 stop-if-true
          w232 = 0.0 ("moteur gauche vite")
          n59 = call "Sous_VI_moteurs.vi"("error in (no error)"=w231, "Moteur Droit"=w232, "Moteur Gauche"=w232) -> ("error out"=w230:errorcluster)  [unwired: 8 in]
          n60 = Less?(x=2000, y=w235) -> (x < y?=w233:bool)
        }
        n61 = call "Labview_trieur_balles.vi"("error in (no error)"=w226) -> ("error out"=w225:errorcluster)  [unwired: 10 in]
      }
      frame "Bras 2" {
        # "Bras en position pour les clapets"
        n62 = while {
          shift-right: [w240] -> w236
          shift-left: w237 -> [w241]
          i -> [w242]
          stop <- w244 stop-if-true
          n63 = Greater Or Equal?(x=w242, y=100000) -> (x >= y?=w245:bool)
          n64 = case shown="False" w245 {
            tunnel: [FALSE TRUE] -> w244
            tunnel: w241 -> [w247 w250]
            tunnel: [w246 w250] -> w240
            frame False {
              n65 = call "Sous_VI_Bras.vi"("error in (no error)"=w247, "Enum bras"=enum_bras."Clapet Bras") -> ("error out"=w246:errorcluster)  [unwired: 9 in]
            }
            frame True {
            }
          }
        }
      }
      frame "Intersection" {
        # "Ignorer la ligne de droite"
        n66 = call "Sous_VI_acq_ligne.vi"("Seuil"=150, "error in (no error)"=w252) -> ("Décalage"=w262:u32, "G/D ?"=w255:bool, "error out"=w253:errorcluster)  [unwired: 8 in, 3 out]
        n67 = call "Sous_VI_correction.vi"("error in (no error)"=w253, "G/D ?"=w255, "Décalage"=w262) -> ("error out"=w254:errorcluster)  [unwired: 8 in]
        n68 = Select(t=Commande_1."Clapet 2", s=w258, f=Commande_1."Intersection") -> (s? t:f=w257:T2)
      }
      frame "Clapet 2" {
        # "Avance en faisant tomber les clapets avec le bras"
        n69 = call "Sous_VI_acq_ligne.vi"("Seuil"=150, "error in (no error)"=w263) -> ("Décalage"=w272:u32, "G/D ?"=w266:bool, "error out"=w264:errorcluster)  [unwired: 8 in, 3 out]
        n70 = call "Sous_VI_correction.vi"("error in (no error)"=w264, "G/D ?"=w266, "Décalage"=w272) -> ("error out"=w265:errorcluster)  [unwired: 8 in]
        n71 = Select(t=Commande_1."Virage 3", s=w267, f=Commande_1."Clapet 2") -> (s? t:f=w268:T2)
      }
      frame "Virage 3" {
        # "Remonte le bras et effectue un virage"
        n72 = while {
          shift-right: [w292] -> w276
          shift-left: w277 -> [w293]
          i -> [w296]
          stop <- w295 stop-if-true
          w294 = 0.0 ("moteur gauche vite")
          n73 = call "Sous_VI_moteurs.vi"("error in (no error)"=w293, "Moteur Droit"=w294, "Moteur Gauche"=w294) -> ("error out"=w292:errorcluster)  [unwired: 8 in]
          n74 = Less?(x=100000, y=w296) -> (x < y?=w295:bool)
        }
        n75 = while {
          shift-right: [w280] -> w275
          shift-left: w276 -> [w281]
          i -> [w282]
          stop <- w284 stop-if-true
          n76 = Greater Or Equal?(x=w282, y=100000) -> (x >= y?=w285:bool)
          n77 = case shown="False" w285 {
            tunnel: [FALSE TRUE] -> w284
            tunnel: w281 -> [w287 w290]
            tunnel: [w286 w290] -> w280
            frame False {
              n78 = call "Sous_VI_Bras.vi"("error in (no error)"=w287, "Enum bras"=enum_bras."Inactif Bras") -> ("error out"=w286:errorcluster)  [unwired: 9 in]
            }
            frame True {
            }
          }
        }
        n79 = call "Sous_VI_Virage_1.vi"("error in (no error)"=w275) -> ("error out"=w274:errorcluster)  [unwired: 10 in]
      }
      frame "Avance" {
        # "Avance jusqu'a la prochaine ligne à droite"
        n80 = call "Sous_VI_acq_ligne.vi"("Seuil"=150, "error in (no error)"=w298) -> ("Décalage"=w303:u32, "G/D ?"=w301:bool, "error out"=w299:errorcluster)  [unwired: 8 in, 3 out]
        n81 = call "Sous_VI_correction.vi"("error in (no error)"=w299, "G/D ?"=w301, "Décalage"=w303) -> ("error out"=w300:errorcluster)  [unwired: 8 in]
        n82 = Select(t=Commande_1."Virage 4", s=w304, f=Commande_1."Avance") -> (s? t:f=w305:T2)
      }
      frame "Virage 4" {
        # "Effectue un virage"
        n83 = call "Sous_VI_Virage_1.vi"("error in (no error)"=w309) -> ("error out"=w310:errorcluster)  [unwired: 10 in]
      }
      frame "Lanceur" {
        # "Se place en position devant la cible, met en route le moteur\nde la roue qui lance les balles puis le moteur du distributeur\npour lancer les balles sur la cible \nEteint les moteur"
        n84 = call "Sous_VI_Lanceur.vi"("error in (no error)"=w313) -> ("error out"=w314:errorcluster)  [unwired: 10 in]
      }
      frame "End" {
        # "Fin du programme"
      }
    }
    "Cluster 3" <- w25
    "Énum 2" <- w31
    n85 = node-c288(w8) -> ()  [unwired: 1 out]
  }
  n86 = node-c288(w5) -> (→"Erreur":errorcluster)
